vi "VI Helpeks Help.vi"   [LabVIEW 2014]
doc: "::: VI Helpeks :::\nCopyright (c) 2000-2026 Konstantin Shifershteyn. All rights reserved."
panel:
  # "VI Helpeks Help"
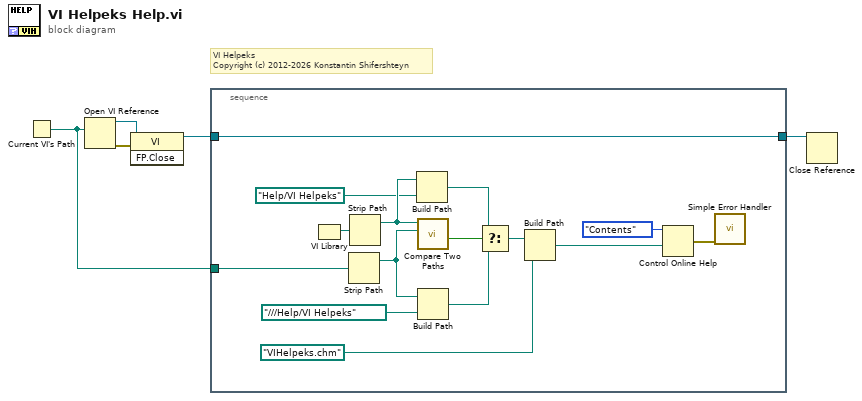
[diagram p0: block diagram]
diagram:
  # "VI Helpeks\nCopyright (c) 2012-2026 Konstantin Shifershteyn"
  n1 = Current VI's Path() -> (path=w1:path)
  n2 = Open VI Reference(vi path=w1) -> (vi reference=w4:refnum<vi>, error out=w5:errorcluster)  [unwired: 5 in]
  n3 = invoke class="VI" method="FP.Close"(reference=w4, error in=w5) -> (reference out=w3:refnum<vi>)  [unwired: 1 in, 2 out]
  n4 = stacked-sequence {
    tunnel: [w20] -> w2
    tunnel: w3 -> [w20]
    tunnel: w1 -> [w17]
    frame #0 {
      n5 = VI Library() -> (path=w18:path)
      n6 = Strip Path(path=w17) -> (stripped path=w9:path)  [unwired: 1 out]
      n7 = Strip Path(path=w18) -> (stripped path=w15:path)  [unwired: 1 out]
      n8 = Build Path(base path=w15, name or relative path=path "Help/VI Helpeks") -> (appended path=w12:path)
      n9 = call <vilib>:"Compare Two Paths.vi"("Path 2"=w9, "Path 1"=w15) -> ("Path 2 Relative to Path 1?"=w16:bool)  [unwired: 6 in, 3 out]
      n10 = Build Path(base path=w9, name or relative path=path "../../../Help/VI Helpeks") -> (appended path=w7:path)
      n11 = Select(t=w12, s=w16, f=w7) -> (s? t:f=w14:path)
      n12 = Build Path(base path=w14, name or relative path=path "VIHelpeks.chm" ("append path")) -> (appended path=w13:path)
      n13 = Control Online Help(2:w13, 4:enum16{"Contents", "Key", "Close"}."Contents" ("Operation")) -> (0:w19:errorcluster)  [unwired: 2 in]
      n14 = call <vilib>:"Simple Error Handler.vi"("error in (no error)"=w19) -> ()  [unwired: 4 in, 5 out]
    }
  }
  n15 = Close Reference(reference=w2) -> ()  [unwired: 1 in, 1 out]
